vi "Data Collection and Save.vi"(7 "CSM Name":string="Data Collection") -> ()   [LabVIEW 2026, in "Data Collection and Save.lvlib"]
uses:
  Data Collection and Save.lvlib
  Supports/Saving States.ctl
  a89fe48b-4482-43cb-96bd-32483feba248.vi
  115e6d42-36e9-43ba-916e-ce7a01ad014e.vi
  adca8abf-46f5-4539-9d33-3f3b2a323202.vi
  ca7f3cfa-0f2a-41ea-9b26-bce09b64ebef.vi
  b5cc49b7-9397-48e9-91c5-f9ab6ae137c5.vi
  eabdaa19-4c7a-45d4-a202-ab5b619048cc.vi
  94bfd1e9-2896-4ece-95aa-b4a38b10d538.vi
  2868361d-398a-4950-9d8e-d0481113e34b.vi
  74be65fa-d069-47f2-ae0a-2e3cfef6bdd0.vi
  <userlib>/_NEVSTOP/Communicable State Machine(CSM)/AdvanceAPI/CSM - Revert Arguments-Safe String.vi
  <userlib>/_NEVSTOP/Communicable State Machine(CSM)/_Shared/Trim Single-line Text.vi
  <userlib>/_NEVSTOP/Communicable State Machine(CSM)/AdvanceAPI/CSM - Make String Arguments Safe.vi
  <userlib>/_NEVSTOP/Communicable State Machine(CSM)/AdvanceAPI/CSM - Break Down Multiple States String.vi
  <userlib>/_NEVSTOP/Communicable State Machine(CSM)/AdvanceAPI/CSM - Compact Multiple States.vi
  <userlib>/_NEVSTOP/Communicable State Machine(CSM)/AdvanceAPI/CSM - Keywords.vi
  <userlib>/_NEVSTOP/Communicable State Machine(CSM)/addons/API-String-Arugments-Support/_Support/Convert API String Arguments to Data(variant).vi
  <userlib>/_NEVSTOP/Communicable State Machine(CSM)/addons/MassData-Parameter/_support/FGV-MassData(lvlibp).vi
  <vilib>/Utility/file.llb/Write To Spreadsheet File (string).vi
  <vilib>/Utility/file.llb/Write To Spreadsheet File (DBL).vi
  <userlib>/_NEVSTOP/Communicable State Machine(CSM)/Communicable State Machine.lvlib
  <userlib>/_NEVSTOP/Communicable State Machine(CSM)/addons/Loop-Support/CSM Loop Support.lvlib
  <userlib>/_NEVSTOP/Communicable State Machine(CSM)/addons/Logger/CSM File Logger.lvlib
panel:
  in  "Exit":bool
  out "Error Occurred":errorcluster
  out "State History":string
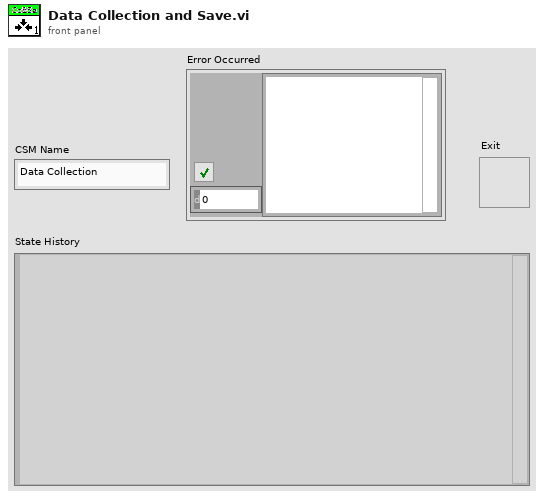
[diagram p1: front panel]
types:
  T1 = enum32{"Invalid", "Standard", "Closed", "Hidden", "Minimized", "Maximized"}
  T2 = enum32{"invalid app kind", "Development System", "Run Time System", "Student Edition", "Embedded LabVIEW", "Evaluation", "Custom"}
  T3 = typedef "温度保存信息.ctl" = cluster{"温度保存-时间":string, "合并保存？":bool, "保存路径":path, "Intervals":dbl}
  T4 = typedef "Data Collection and Save.lvlib/Saving States.ctl" = enum16{"Idle", "Saving", "Error"}
  T5 = typedef "Communicable State Machine.lvlib/_CSM_Response Source Message.ctl" = cluster{"‘State":string, "’Arguments":string, "’Error":errorcluster}
  T6 = cluster{"Current VI Reference":refnum<vi>, "Close Panel on Exit?":bool}
  T7 = typedef "全局变量数据.ctl" = cluster{"温度采集":dbl[], "温度控制":dbl[], "压力测量":dbl[], "Zolix":dbl[], "步进电机":dbl[], "湿度测量":dbl[], "距离测量":dbl[]}
  T8 = cluster{"Core":cluster{"Current VI Reference":refnum<vi>, "Close Panel on Exit?":bool}, "State":T4, "数据及Titles":cluster{"Titles":string[], "温度相关数据":T7}, "文件保存信息":cluster{"温度数据保存文件-时间":string, "合并保存？":bool, "BasePath":path, "Intervals":dbl}, "自停标志":cluster{"接收数":u32, "停止次数":u32, "interval 备份":dbl, "采集时间":timestamp}}
  T9 = cluster{"接收数":u32, "停止次数":u32, "interval 备份":dbl, "采集时间":timestamp}
  T10 = cluster{"温度数据保存文件-时间":string, "合并保存？":bool, "BasePath":path, "Intervals":dbl}
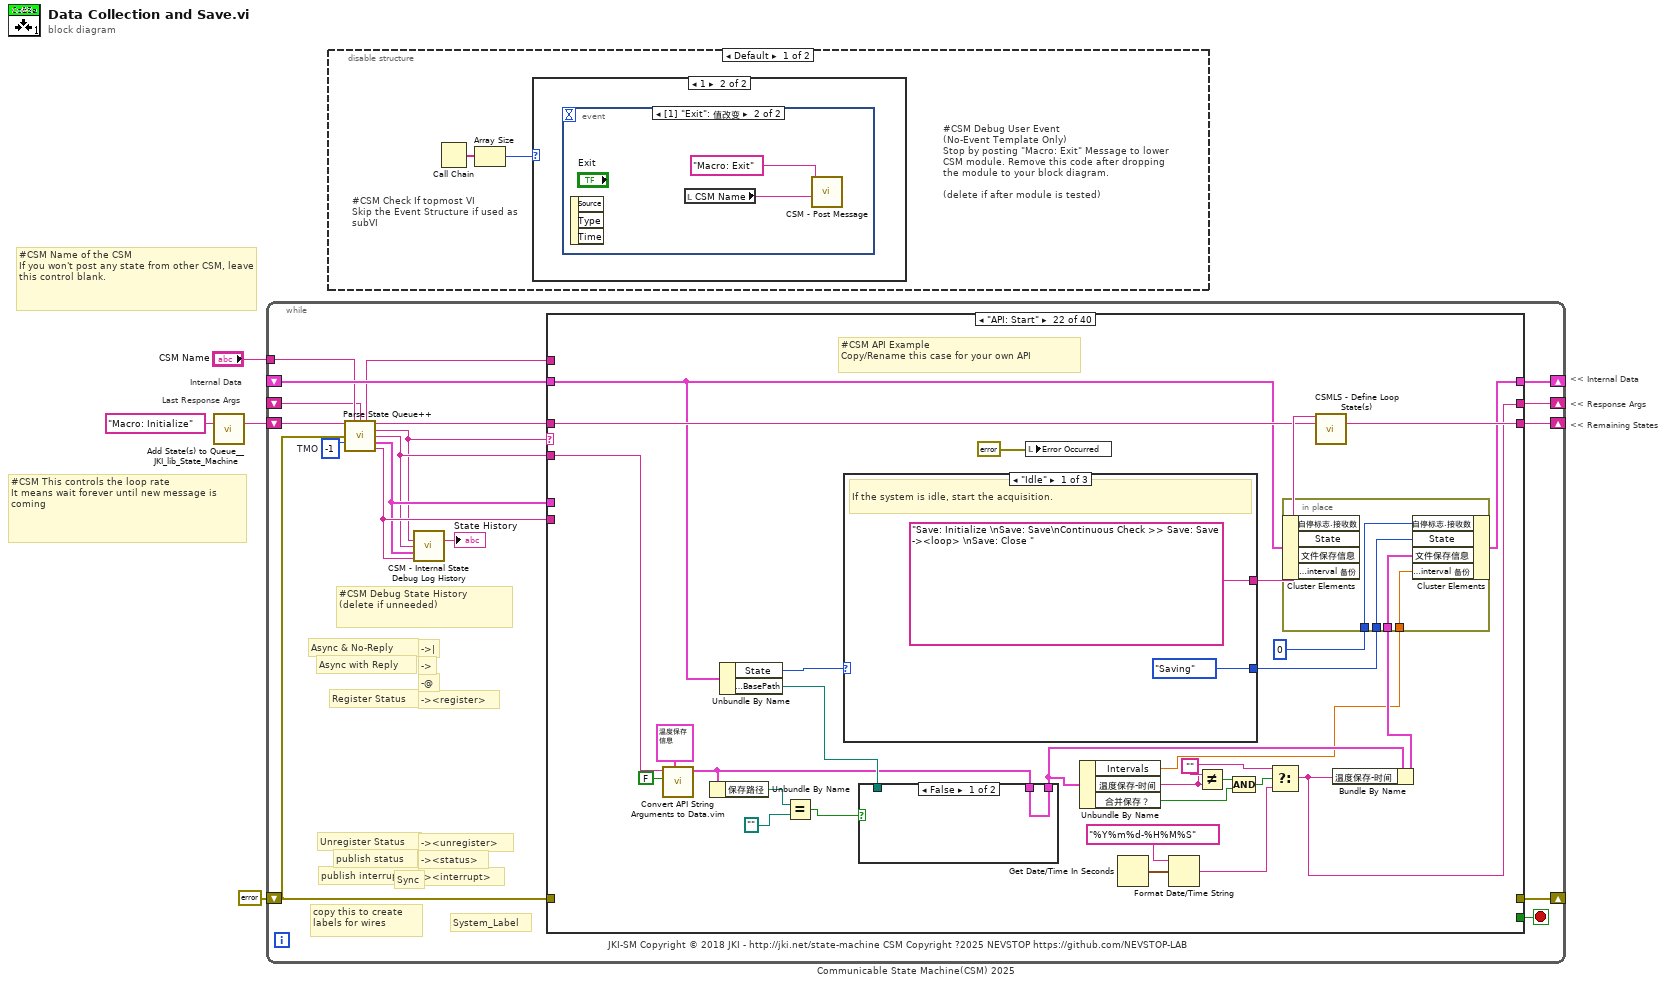
[diagram p0: block diagram]
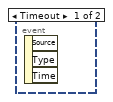
[diagram p3: hidden frame]
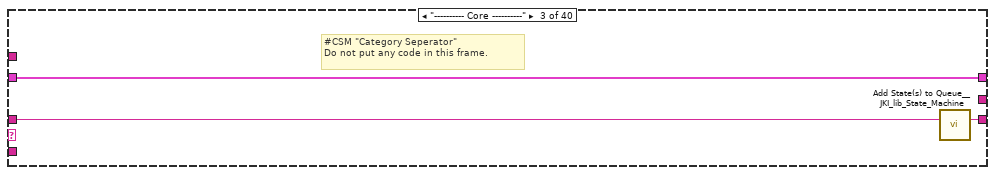
[diagram p7: hidden frame]
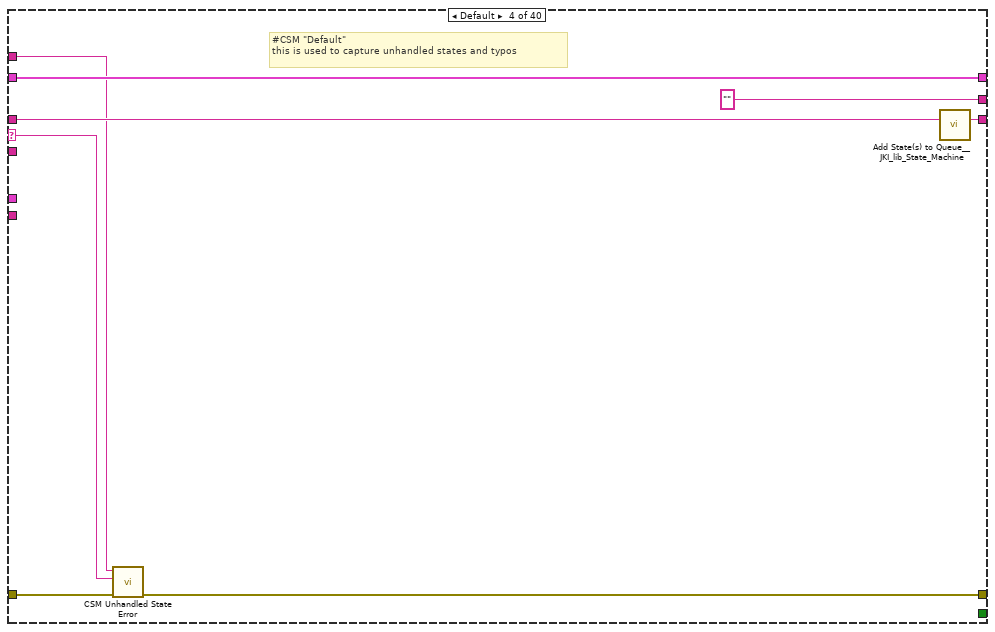
[diagram p8: hidden frame]
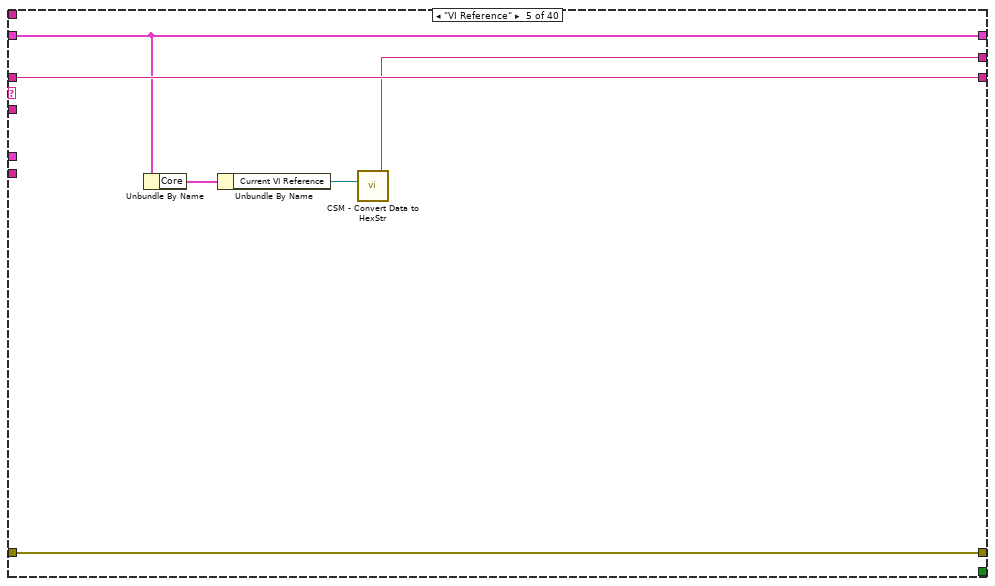
[diagram p9: hidden frame]
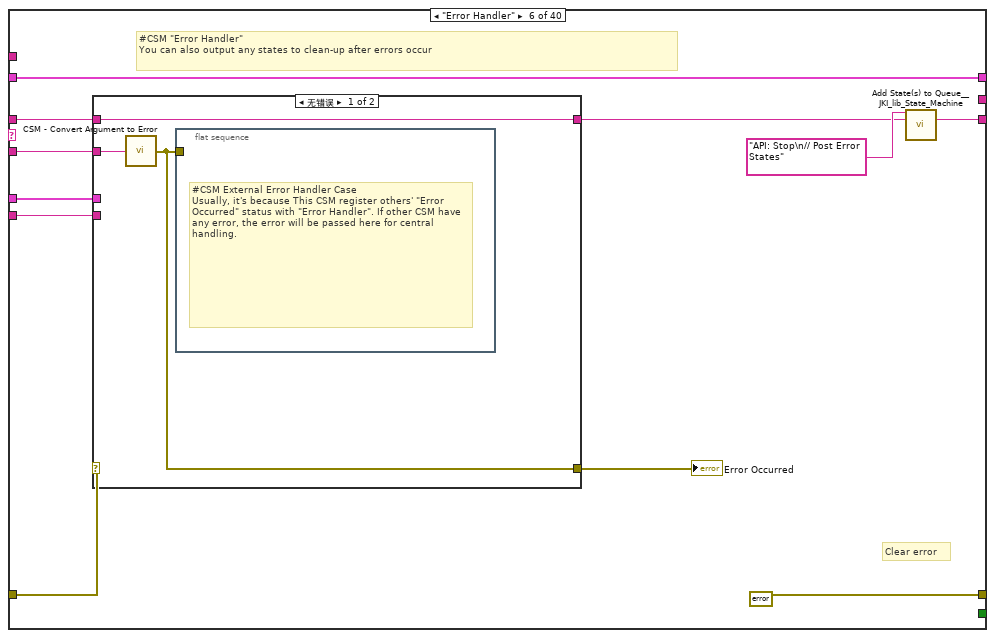
[diagram p10: hidden frame]
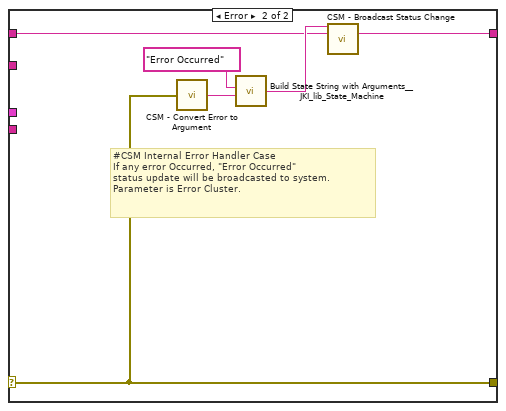
[diagram p11: hidden frame]
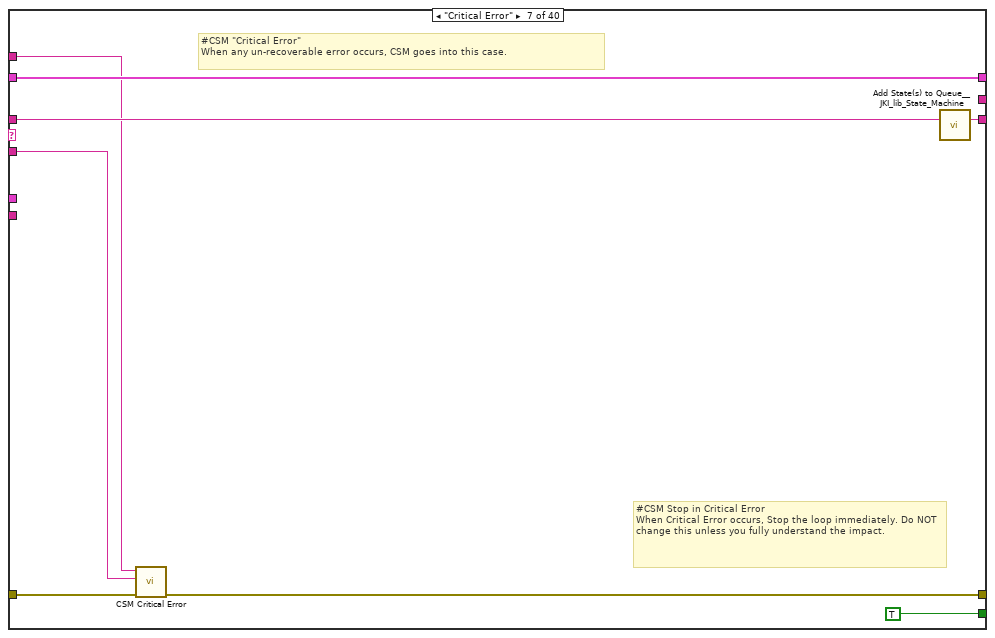
[diagram p12: hidden frame]
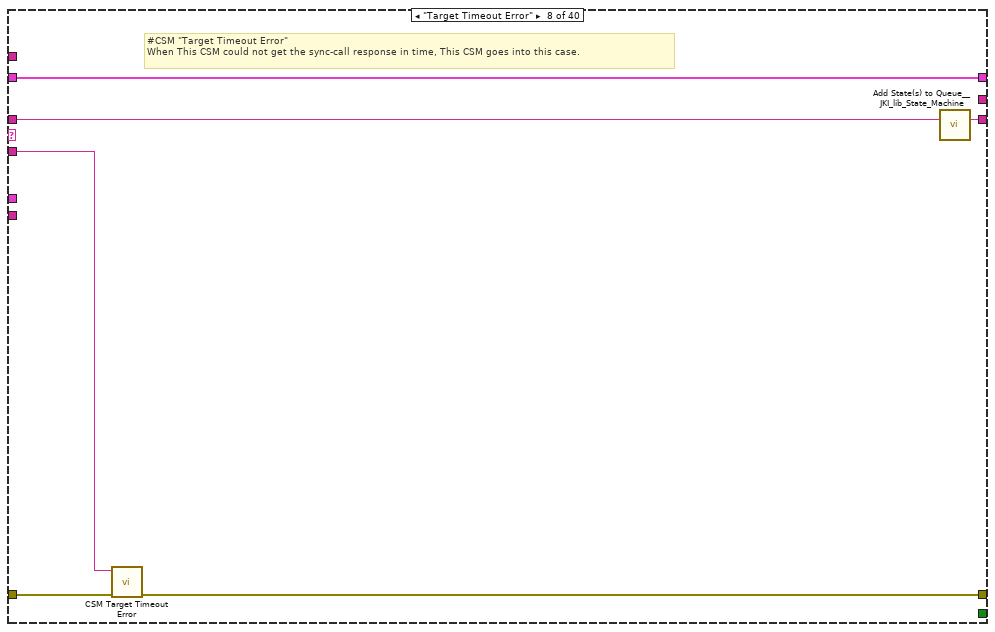
[diagram p13: hidden frame]
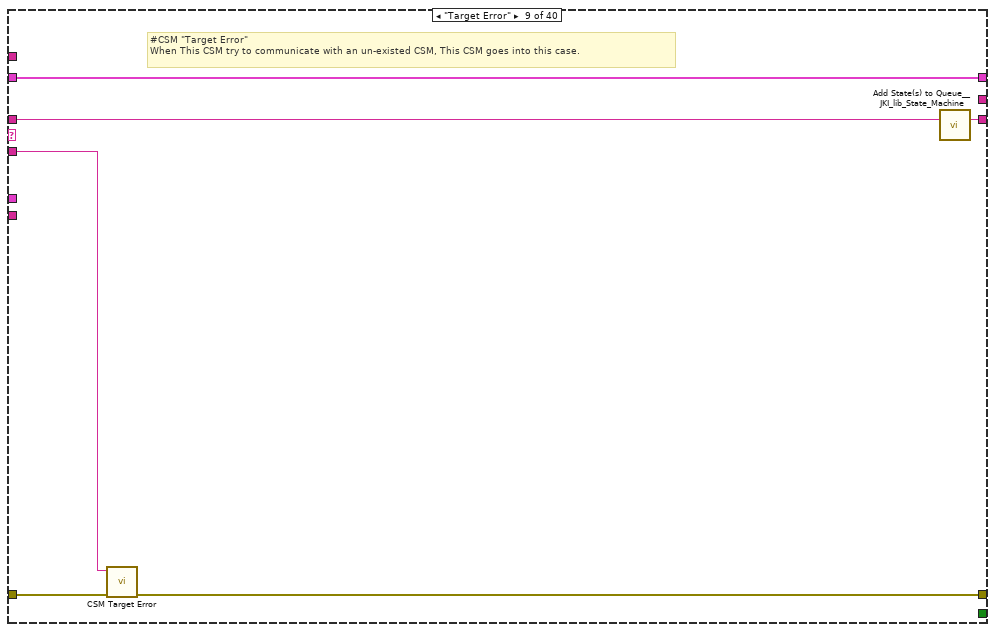
[diagram p14: hidden frame]
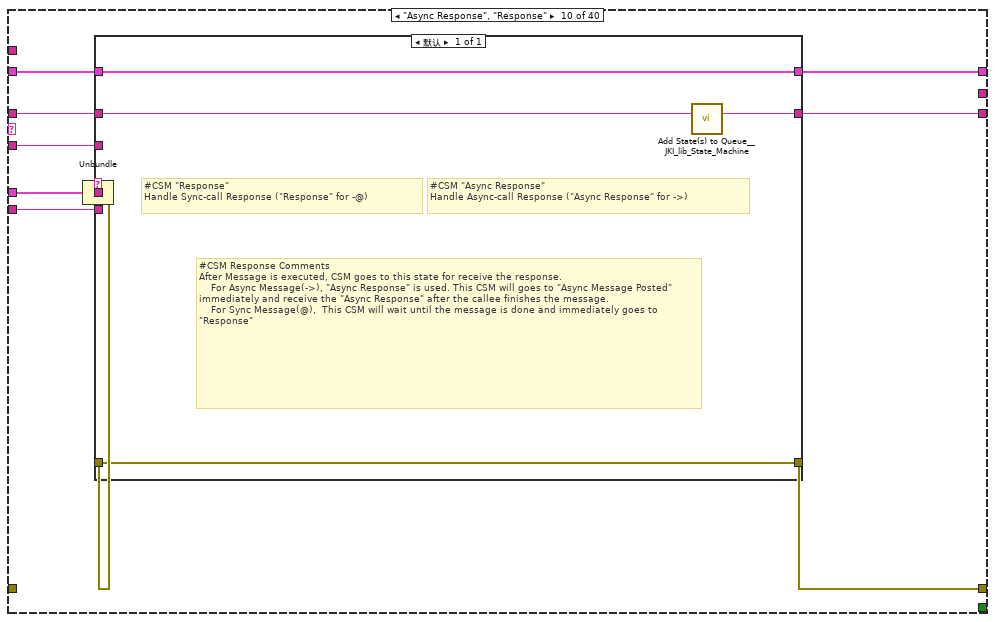
[diagram p15: hidden frame]
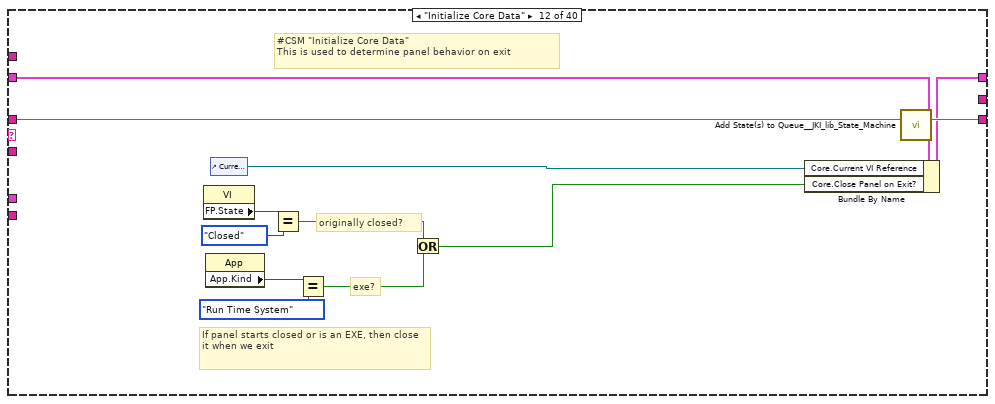
[diagram p17: hidden frame]
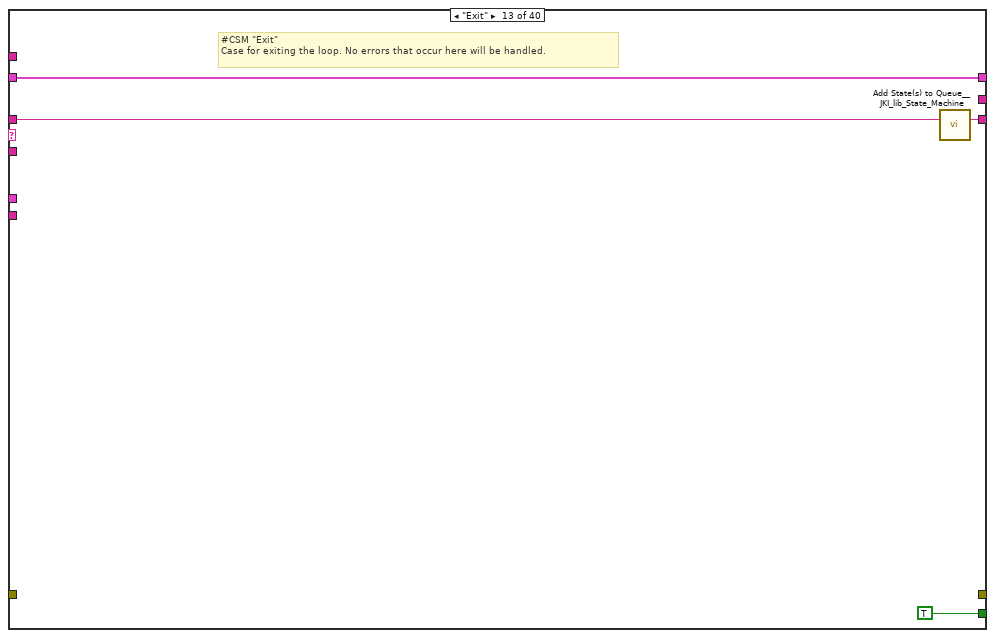
[diagram p18: hidden frame]
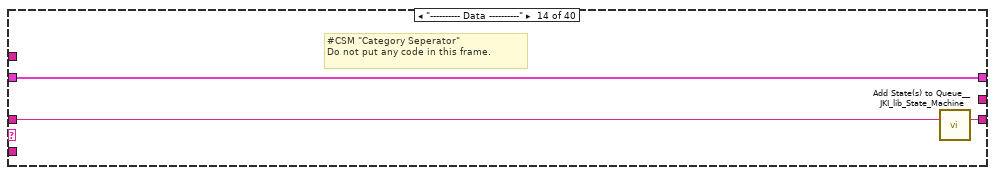
[diagram p19: hidden frame]
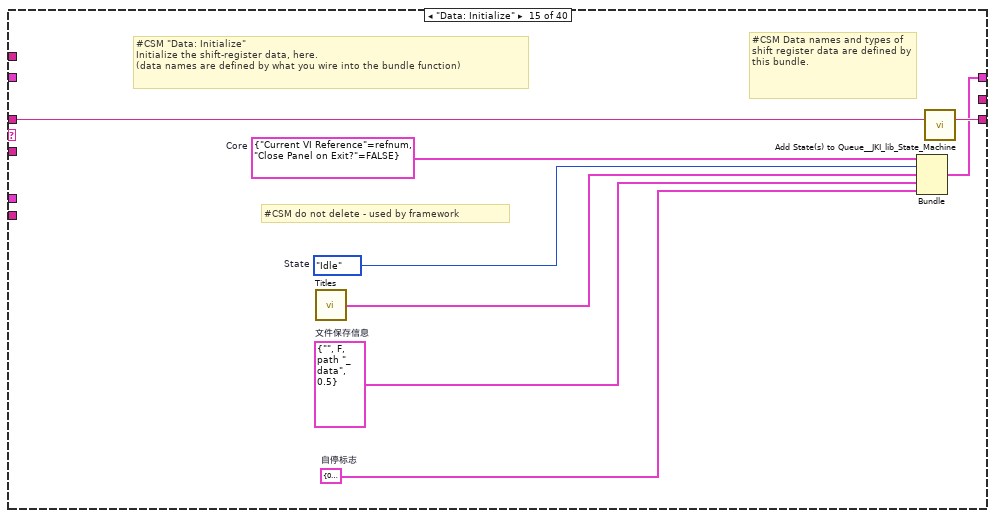
[diagram p20: hidden frame]
diagram:
  # "Last Response Args"
  # "Internal Data"
  # "#CSM Name of the CSM\nIf you won't post any state from other CSM, leave this control blank."
  # "#CSM This controls the loop rate\nIt means wait forever until new message is coming"
  # "<< Internal Data"
  # "<< Response Args"
  # "<< Remaining States"
  n1 = call <vilib>:"Add State(s) to Queue__JKI_lib_State_Machine.vi"("State(s) in (\"\")"="Macro: Initialize" ("Init State(\"Macro: Initialize\")")) -> ("States Out"=w1:string)  [unwired: 14 in]
  n2 = while "Communicable State Machine(CSM) 2025" {
    shift-right: [w17] -> _
    shift-left: _ -> [w16]
    shift-right: [w20] -> _
    shift-left: errorcluster {"status"=FALSE, "code"=0, "source"=""} ("error out") -> [w6]
    shift-right: [w19] -> _
    shift-left: w1 -> [w21]
    tunnel: "CSM Name" -> [w13]
    shift-right: [w14] -> _
    shift-left: _ -> [w8]
    stop <- w18 stop-if-true
    w15 = -1  # TMO
    # "#CSM Debug State History\n(delete if unneeded)"
    # "-><interrupt>"
    # "-><status>"
    # "-><unregister>"
    # "-><register>"
    # "-@"
    # "->"
    # "->|"
    # "publish interrupt"
    # "publish status"
    # "Unregister Status"
    # "Register Status"
    # "Sync"
    # "Async with Reply"
    # "Async & No-Reply"
    # "JKI-SM Copyright © 2018 JKI - http://jki.net/state-machine CSM Copyright ?2025 NEVSTOP https://github.com/NEVSTOP-LAB"
    # "copy this to create labels for wires"
    # "System_Label"
    n3 = call <userlib>:"Parse State Queue++.vi"("State Queue"=w21, "Name (\"\" to Use UUID)"=w13, "Response Arguments"=w8, "Previous Error"=w6, "Dequeue (1 ms)"=w15) -> ("Name Used"=w7:string, "Remaining States"=w22:string, "Current State"=w9:string, "Arguments"=w10:string, "Additional Information"=w11:T5, "Source CSM"=w12:string)  [unwired: 5 in]
    n4 = call <userlib>:"CSM - Internal State Debug Log History.vi"("State"=w9, "Arguments (\"\")"=w10, ">> Response Source Message >>"=w11, "Source (\"\")"=w12) -> ("Debug Log"=→"State History":string)  [unwired: 11 in]
    n5 = case shown="\"API: Start\"" w9 {
      selector: w9 -> [_ _ _ w33 _ _ _ _ _ _ _ _ _ _ _ _ _ _ _ _ _ _ _ _ _ _ _ _ _ _ _ _ _ _ _ _ _ _ w400 _]
      tunnel: w22 -> [w23 w26 w29 w37 w42 w48 w71 w77 w83 w93 w100 w112 w116 w119 w127 w130 w136 w139 w143 w151 w156 w184 w203 w214 w218 w228 w240 w252 w264 w276 w288 w300 w305 w318 w330 w365 w370 w374 w401 w406]
      tunnel: w10 -> [_ _ _ _ _ w47 w67 w74 w80 w87 _ _ _ _ _ _ _ _ _ _ _ w181 _ w212 _ w226 w237 w249 w260 w272 w284 w296 _ _ _ _ _ _ w398 _]
      tunnel: w16 -> [w24 w25 w27 w35 w41 w53 w69 w75 w81 w91 w99 w106 w114 w117 _ w128 w131 w137 w141 w147 w157 w163 w204 w210 w216 w222 w234 w246 w258 w270 w282 w294 w303 w309 w326 w363 w367 w372 w378 w405]
      tunnel: [_ _ _ w30 w43 errorcluster {"status"=FALSE, "code"=0, "source"=""} ("error out") w64 w72 w78 w94 _ _ _ _ _ _ w132 _ _ _ _ _ _ _ _ _ _ _ _ _ _ _ _ w310 w332 _ _ _ _ w407] -> w20
      tunnel: w6 -> [_ _ _ w31 w43 w51 w65 w73 w79 _ _ _ _ _ _ _ w133 _ _ _ _ _ _ _ _ _ _ _ _ _ _ _ _ _ w333 _ _ _ _ w407]
      tunnel: [w23 w26 w28 w36 w42 w49 w70 w76 w82 w92 w100 w111 w115 w118 w126 w130 w135 w138 w142 w150 w155 w183 w202 w213 w217 w227 w239 w251 w263 w275 w287 w299 w304 w318 w331 w364 w369 w373 w399 w404] -> w19
      tunnel: [_ _ _ _ _ _ TRUE _ _ _ _ _ TRUE _ _ _ _ _ _ _ _ _ _ _ _ _ _ _ _ _ _ _ _ _ _ _ _ _ _ _] -> w18
      tunnel: [w24 w25 w27 w35 w41 w53 w69 w75 w81 w90 w99 w110 w114 w117 w125 w128 w131 w137 w141 w147 w157 w162 w204 w209 w216 w221 w233 w245 w257 w269 w281 w291 w303 w308 w329 w363 w366 w372 w377 w405] -> w17
      tunnel: w12 -> [_ _ _ _ _ w46 _ _ _ w88 _ _ _ _ _ _ _ _ _ _ _ _ _ _ _ _ _ _ _ _ _ _ _ _ _ _ _ _ _ _]
      tunnel: w11 -> [_ _ _ _ _ w45 _ _ _ w89 _ _ _ _ _ _ _ _ _ _ _ _ _ _ _ _ _ _ _ _ _ _ _ _ _ _ _ _ _ _]
      tunnel: [_ _ _ "" w38 _ _ _ _ _ _ _ _ _ _ _ _ _ _ _ _ w166 _ _ _ _ _ _ _ _ _ _ _ _ _ _ _ _ _ _] -> w14
      tunnel: w7 -> [_ _ _ w32 _ _ w66 _ _ _ _ _ _ _ _ _ _ _ _ _ _ _ _ _ _ _ _ _ _ _ _ _ _ _ _ _ _ _ _ _]
      frame "", "Idle" {
        # "#CSM \"Idle/Event Handler\"\nexecutes when the state queue is empty"
      }
      frame "CSM Documentation" {
        # "#CSM State Syntax\n\n// Comment line, all text to the right of “//” will be ignored\n// Local Message Example\nDoSth: DoA >> Arguments\n\n// Sync Call Example\nAPI: xxxx >> Arguments -@ TargetModule\n\n// Async Call Example\nAPI: xxxx >> Arguments -> TargetModule\n\n// Async Call without Reply Example\nAPI: xxxx >> Arguments ->| TargetModule\n\n// Broadcast normal status:\nStatus >> StatusArguments  -><status>\n\n// Broadcast Interrupt status:\nInterrupt >> StatusArguments  -><interrupt>\n\n// Register Source Module's status to Handler Module\nStatus@Source Module >> Handler Module@Handler Module -><register>\n\n// Unegister Source Module's status\nStatus@Source Module >> Handler Module -><unregister>"
        # "#CSM README FIRST\n\nCommunicable State Machine(CSM) is a LabVIEW application framework that builds upon JKI State Machine(JKISM). It follows the pattern of JKISM and extends the keywords to describe message communication between modules, including concepts such as Sync-Message, Async-Message, Subscription/Unsubscription of status - essential elements for creating reusable code modules. For more information, please visit the CSM wiki: https://nevstop-lab.github.io/CSM-Wiki/\n\nFor instructions on JKI State Machine, visit: \n    http://jki.net/state-machine/\nFor information about CSM, visit: \n    https://github.com/NEVSTOP-LAB"
        # "#CSM \"Documentation\"\nCase for holding CSM Documenation"
      }
      frame "---------- Core ----------" {
        # "#CSM \"Category Seperator\"\nDo not put any code in this frame."
        n6 = call <vilib>:"Add State(s) to Queue__JKI_lib_State_Machine.vi"("State(s) in (\"\")"=w29) -> ("States Out"=w28:string)  [unwired: 14 in]
      }
      frame Default {
        # "#CSM \"Default\"\nthis is used to capture unhandled states and typos"
        n7 = call <userlib>:"CSM Unhandled State Error.vi"("error in (no error)"=w31, "Undefined State"=w33, "CSM Name"=w32) -> ("error out"=w30:errorcluster)  [unwired: 8 in]
        n8 = call <vilib>:"Add State(s) to Queue__JKI_lib_State_Machine.vi"("State(s) in (\"\")"=w37) -> ("States Out"=w36:string)  [unwired: 14 in]
      }
      frame "VI Reference" {
        n9 = Unbundle By Name(w41) -> ("Core"=w40:T6)
        n10 = Unbundle By Name(w40) -> ("Current VI Reference"=w39:refnum<vi>)
        n11 = call <userlib>:"CSM - Convert Data to HexStr.vi"("Variant"=w39) -> ("HEX String (0-9,A-F)"=w38:string)  [unwired: 8 in]
      }
      frame "Error Handler" {
        # "#CSM \"Error Handler\"\nYou can also output any states to clean-up after errors occur"
        # "Clear error"
        n12 = case shown="无错误" w51 {
          selector: w51 -> [_ w58]
          tunnel: [w57 w60] -> w50
          tunnel: w48 -> [w57 w59]
          tunnel: w47 -> [w56 _]
          tunnel: w46 -> [_ _]
          tunnel: w45 -> [_ _]
          tunnel: [w55 w58] -> w44
          frame No Error {
            n13 = call <userlib>:"CSM - Convert Argument to Error.vi"("Argument"=w56) -> ("Error"=w55:errorcluster)  [unwired: 4 in]
            n14 = flat-sequence {
              tunnel: w55 -> [_]
              frame #0 {
                # "#CSM External Error Handler Case\nUsually, it's because This CSM register others' \"Error Occurred\" status with \"Error Handler\". If other CSM have any error, the error will be passed here for central handling."
              }
            }
          }
          frame Error {
            # "#CSM Internal Error Handler Case \nIf any error Occurred, \"Error Occurred\" \nstatus update will be broadcasted to system.\nParameter is Error Cluster."
            n15 = call <userlib>:"CSM - Convert Error to Argument.vi"("Error"=w58) -> ("Argument"=w62:string)  [unwired: 4 in]
            n16 = call <vilib>:"Build State String with Arguments__JKI_lib_State_Machine.vi"("Arguments (\"\")"=w62, "State"="Error Occurred" ("Status with Arguments")) -> ("State with Arguments"=w61:string)  [unwired: 4 in]
            n17 = call <userlib>:"CSM - Broadcast Status Change.vi"("Status With Arguments"=w61, "State Queue"=w59) -> ("Remaining States"=w60:string)  [unwired: 13 in]
          }
        }
        "Error Occurred" <- w44
        n18 = call <vilib>:"Add State(s) to Queue__JKI_lib_State_Machine.vi"("State(s) in Front (\"\")"="API: Stop\n// Post Error States", "State(s) in (\"\")"=w50) -> ("States Out"=w49:string)  [unwired: 13 in]
      }
      frame "Critical Error" {
        # "#CSM \"Critical Error\"\nWhen any un-recoverable error occurs, CSM goes into this case."
        # "#CSM Stop in Critical Error\nWhen Critical Error occurs, Stop the loop immediately. Do NOT change this unless you fully understand the impact."
        n19 = call <userlib>:"CSM Critical Error.vi"("error in (no error)"=w65, "Arugments (As Reason)"=w67, "CSM Name"=w66) -> ("error out"=w64:errorcluster)  [unwired: 8 in]
        n20 = call <vilib>:"Add State(s) to Queue__JKI_lib_State_Machine.vi"("State(s) in (\"\")"=w71) -> ("States Out"=w70:string)  [unwired: 14 in]
      }
      frame "Target Timeout Error" {
        # "#CSM \"Target Timeout Error\"\nWhen This CSM could not get the sync-call response in time, This CSM goes into this case."
        n21 = call <userlib>:"CSM Target Timeout Error.vi"("error in (no error)"=w73, "Arguments (As CSM Name)"=w74) -> ("error out"=w72:errorcluster)  [unwired: 9 in]
        n22 = call <vilib>:"Add State(s) to Queue__JKI_lib_State_Machine.vi"("State(s) in (\"\")"=w77) -> ("States Out"=w76:string)  [unwired: 14 in]
      }
      frame "Target Error" {
        # "#CSM \"Target Error\"\nWhen This CSM try to communicate with an un-existed CSM, This CSM goes into this case."
        n23 = call <userlib>:"CSM Target Error.vi"("error in (no error)"=w79, "Arguments (As CSM Name)"=w80) -> ("error out"=w78:errorcluster)  [unwired: 9 in]
        n24 = call <vilib>:"Add State(s) to Queue__JKI_lib_State_Machine.vi"("State(s) in (\"\")"=w83) -> ("States Out"=w82:string)  [unwired: 14 in]
      }
      frame "Async Response", "Response" {
        n25 = Unbundle(w89) -> ("‘State"=w86:string, "’Arguments"=w85:string, "’Error"=w84:errorcluster)
        n26 = case shown="默认" w86 {
          tunnel: [w95] -> w92
          tunnel: w93 -> [w96]
          tunnel: [w98] -> w90
          tunnel: w91 -> [w98]
          tunnel: [w97] -> w94
          tunnel: w84 -> [w97]
          tunnel: w88 -> [_]
          tunnel: w87 -> [_]
          tunnel: w85 -> [_]
          frame 默认 {
            # "#CSM \"Async Response\"\nHandle Async-call Response (\"Async Response\" for ->)"
            # "#CSM \"Response\"\nHandle Sync-call Response (\"Response\" for -@)"
            # "#CSM Response Comments\nAfter Message is executed, CSM goes to this state for receive the response.\n    For Async Message(->), \"Async Response\" is used. This CSM will goes to \"Async Message Posted\" immediately and receive the \"Async Response\" after the callee finishes the message.\n    For Sync Message(@),  This CSM will wait until the message is done and immediately goes to \"Response\""
            n27 = call <vilib>:"Add State(s) to Queue__JKI_lib_State_Machine.vi"("State(s) in (\"\")"=w96) -> ("States Out"=w95:string)  [unwired: 14 in]
          }
        }
      }
      frame "Async Message Posted" {
        # "#CSM \"Async Message Posted\"\nAfter Async Message is posted (-> or ->| ), CSM goes to this state for post-action.\nYou can use Argument - State to tell which Async Message is called."
      }
      frame "Initialize Core Data" {
        # "#CSM \"Initialize Core Data\"\nThis is used to determine panel behavior on exit"
        # "originally closed?"
        # "exe?"
        # "If panel starts closed or is an EXE, then close it when we exit"
        n28 = property class="VI"() -> ("FP.State"=w103:T1)  [unwired: 2 in, 2 out]
        n29 = property class="App"() -> ("App.Kind"=w109:T2)  [unwired: 2 in, 2 out]
        n30 = control-ref of="Current VI Reference"() -> (w104:refnum<vi>)
        n31 = Equal?(x=w103, y=T1."Closed" ("Front Panel Window:State")) -> (x = y?=w101:bool)
        n32 = Equal?(x=w109, y=T2."Run Time System" ("Application:Kind")) -> (x = y?=w107:bool)
        n33 = Or(x=w101, y=w107) -> (x .or. y?=w105:bool)
        n34 = Bundle By Name(cluster=w106, "Core.Current VI Reference"=w104, "Core.Close Panel on Exit?"=w105) -> (w110:T8)
        n35 = call <vilib>:"Add State(s) to Queue__JKI_lib_State_Machine.vi"("State(s) in (\"\")"=w112) -> ("States Out"=w111:string)  [unwired: 14 in]
      }
      frame "Exit" {
        # "#CSM \"Exit\"\nCase for exiting the loop. No errors that occur here will be handled."
        n36 = call <vilib>:"Add State(s) to Queue__JKI_lib_State_Machine.vi"("State(s) in (\"\")"=w116) -> ("States Out"=w115:string)  [unwired: 14 in]
      }
      frame "---------- Data ----------" {
        # "#CSM \"Category Seperator\"\nDo not put any code in this frame."
        n37 = call <vilib>:"Add State(s) to Queue__JKI_lib_State_Machine.vi"("State(s) in (\"\")"=w119) -> ("States Out"=w118:string)  [unwired: 14 in]
      }
      frame "Data: Initialize" {
        w120 = T9 {"接收数"=0, "停止次数"=0, "interval 备份"=0.0, "采集时间"=timestamp(0 s since 1904-01-01)}  # 自停标志
        w122 = T10 {"温度数据保存文件-时间"="", "合并保存？"=FALSE, "BasePath"=path "_data", "Intervals"=0.5}  # 文件保存信息
        w123 = Saving_States."Idle"  # State
        w124 = T6 {"Current VI Reference"=refnum, "Close Panel on Exit?"=FALSE}  # Core
        # "#CSM \"Data: Initialize\"\nInitialize the shift-register data, here.\n(data names are defined by what you wire into the bundle function)"
        # "#CSM do not delete - used by framework"
        # "#CSM Data names and types of shift register data are defined by this bundle."
        n38 = call "Titles.vi"() -> ("数据及Titles"=w121:cluster{"Titles":string[], "温度相关数据":T7})  [unwired: 1 in]
        n39 = Bundle("Core"=w124, "State"=w123, "数据及Titles"=w121, "文件保存信息"=w122, "自停标志"=w120) -> (w125:T8)  [unwired: 1 in]
        n40 = call <vilib>:"Add State(s) to Queue__JKI_lib_State_Machine.vi"("State(s) in (\"\")"=w127) -> ("States Out"=w126:string)  [unwired: 14 in]
      }
      frame "Data: Update Indicators" {
        n41 = local write "Error Occurred"(errorcluster {"status"=FALSE, "code"=0, "source"=""} ("错误常量")) -> ()
      }
      frame "Data: Cleanup" {
        # "#CSM \"Data: Cleanup\"\nCleanup any data and references, here.\n(this is called automatically, by the Macro: Exit)"
        n42 = Unbundle By Name(w131) -> ("Core.Current VI Reference"=w134:refnum<vi>)
        n43 = Close Reference(reference=w134, error in (no error)=w133) -> (error out=w132:errorcluster)
        n44 = call <vilib>:"Add State(s) to Queue__JKI_lib_State_Machine.vi"("State(s) in (\"\")"=w136) -> ("States Out"=w135:string)  [unwired: 14 in]
      }
      frame "---------- Macro ----------" {
        # "#CSM \"Category Seperator\"\nDo not put any code in this frame."
        n45 = call <vilib>:"Add State(s) to Queue__JKI_lib_State_Machine.vi"("State(s) in (\"\")"=w139) -> ("States Out"=w138:string)  [unwired: 14 in]
      }
      frame "Macro: Initialize" {
        # "#CSM \"Macro: Initialize\"\nInitialization Macro (This is called once, when the VI starts)"
        n46 = call <vilib>:"Add State(s) to Queue__JKI_lib_State_Machine.vi"("State(s) in Front (\"\")"="Data: Initialize\nInitialize Core Data\nData: Update Indicators", "State(s) in (\"\")"=w143) -> ("States Out"=w142:string)  [unwired: 13 in]
      }
      frame "Macro: Exit" {
        # "#CSM \"Macro: Exit\"\nExit Macro (This is called once, when the VI exits)"
        n47 = Unbundle By Name(w147) -> ("State"=w146:T4)
        n48 = case shown="\"Saving\"" w146 {
          tunnel: ["" "Break Continuous\nDAQ: Close" ""] -> w144
          frame "Idle", Default {
          }
          frame "Saving" {
          }
          frame "Error" {
          }
        }
        n49 = call <vilib>:"Add State(s) to Queue__JKI_lib_State_Machine.vi"("State(s) in Front (\"\")"="//Exit Sub-Modules ", "State(s) in (\"\")"=w144, "State(s) at Back (\"\")"="Data: Cleanup\nExit") -> ("States Out"=w148:string)  [unwired: 12 in]
        n50 = call <vilib>:"Add State(s) to Queue__JKI_lib_State_Machine.vi"("State(s) in Front (\"\")"=w148, "State(s) in (\"\")"=w151) -> ("States Out"=w150:string)  [unwired: 13 in]
      }
      frame "---------- API ----------" {
        # "#CSM \"Category Seperator\"\nDo not put any code in this frame."
        n51 = call <vilib>:"Add State(s) to Queue__JKI_lib_State_Machine.vi"("State(s) in (\"\")"=w156) -> ("States Out"=w155:string)  [unwired: 14 in]
      }
      frame "API: Start" {
        # "#CSM API Example\nCopy/Rename this case for your own API"
        n52 = call "Convert API String Arguments to Data.vim"("Reference Type"=T3 {"温度保存-时间"="", "合并保存？"=FALSE, "保存路径"=path "D:/sunrise/data", "Intervals"=0.0} ("输出簇"), "Strict Label Check? (T)"=FALSE, "API String"=w181) -> ("Data"=w176:T3)  [unwired: 5 in, 1 out]
        n53 = Unbundle By Name(w176) -> ("保存路径"=w179:path)
        n54 = Unbundle By Name(w163) -> ("State"=w186:T4, "文件保存信息.BasePath"=w178:path)
        n55 = Equal?(x=w179, y=path "") -> (x = y?=w177:bool)
        n56 = case shown="\"Idle\"" w186 {
          selector: w186 -> [_ w199 w200]
          tunnel: [Saving_States."Saving" ("Acquisition State") w199 w200] -> w160
          tunnel: ["Save: Initialize \nSave: Save\nContinuous Check >> Save: Save -><loop> \nSave: Close " ("State(s) in Front (\"\")") _ _] -> w185
          frame "Idle" {
            # "If the system is idle, start the acquisition."
          }
          frame "Saving" {
            # "The system is already acquiring. Ignore the \"Start\" message."
          }
          frame "Error" {
          }
        }
        n57 = case shown="False" w177 {
          tunnel: w178 -> [_ w196]
          tunnel: w176 -> [w191 w195]
          tunnel: [w191 w194] -> w167
          frame False {
          }
          frame True {
            n58 = call <userlib>:"Append CSM AppDir If Relative.vi"("Relative Path (.)"=w196) -> ("Application Directory (+ Relative)"=w193:path)  [unwired: 4 in]
            n59 = call "__MGI Create Directory Chain_CO.vi"("Path"=w193) -> ("Duplicate Path"=w192:path)  [unwired: 9 in, 1 out]
            n60 = Bundle By Name(cluster=w195, "保存路径"=w192) -> (w194:T3)
          }
        }
        n61 = local write "Error Occurred"(errorcluster {"status"=FALSE, "code"=0, "source"=""} ("错误常量")) -> ()
        n62 = Unbundle By Name(w167) -> ("Intervals"=w158:dbl, "温度保存-时间"=w169:string, "合并保存？"=w168:bool)
        n63 = Get Date/Time In Seconds() -> (seconds since 1Jan1904=w173:timestamp)
        n64 = Format Date/Time String(time format string (%c)="%Y%m%d-%H%M%S" ("时间格式字符串(%c)"), seconds (now)=w173) -> (date/time string=w170:string)  [unwired: 1 in]
        n65 = Not Equal?(x="", y=w169) -> (x != y?=w174:bool)
        n66 = Compound Arithmetic op=AND ("复合运算")(w174, w168) -> (w175:bool)
        n67 = Select(t=w169, s=w175, f=w170) -> (s? t:f=w166:string)
        n68 = call <userlib>:"CSMLS - Define Loop State(s).vi"("Loop States"=w185, "States Queue"=w184) -> ("Remaining States"=w183:string)  [unwired: 13 in]
        n69 = Bundle By Name(cluster=w167, "温度保存-时间"=w166) -> (w159:T3)
        n70 = in-place {
          in-place-border: u32 0 ("广播数") -> [w190]
          in-place-border: w160 -> [w189]
          in-place-border: w159 -> [w188]
          in-place-border: w158 -> [w187]
          n71 = in-place-cluster #1(w163) -> ()  [unwired: 4 out]
          n72 = in-place-cluster #1("自停标志.接收数"=w190, "State"=w189, "文件保存信息"=w188, "自停标志.interval 备份"=w187) -> (w162:T8)
        }
      }
      frame "API: Stop" {
        # "#CSM API Example\nCopy/Rename this case for your own API"
        n73 = Unbundle By Name(w204) -> ("State"=w205:T4)
        n74 = case shown="\"Saving\"" w205 {
          tunnel: [_ "Break Continuous" ("State(s) in Front (\"\")") "Break Continuous" ("State(s) in Front (\"\")")] -> w201
          frame "Idle" {
            # "The system is already idle. Ignore the \"Stop\" message."
          }
          frame "Saving" {
            # "If the system is acquiring, stop the acquisition."
          }
          frame "Error" {
          }
        }
        n75 = call <vilib>:"Add State(s) to Queue__JKI_lib_State_Machine.vi"("State(s) in Front (\"\")"=w201, "State(s) in (\"\")"=w203) -> ("States Out"=w202:string)  [unwired: 13 in]
      }
      frame "API: Save Interval" {
        n76 = call "Convert API String Arguments to Data.vim"("Reference Type"=0.0, "API String"=w212) -> ("Data"=w208:dbl)  [unwired: 6 in, 1 out]
        n77 = in-place {
          in-place-border: w208 -> [w215]
          n78 = in-place-cluster #2(w210) -> ()  [unwired: 2 out]
          n79 = in-place-cluster #2("文件保存信息.Intervals"=w215, "自停标志.interval 备份"=w215) -> (w209:T8)
        }
        n80 = call <vilib>:"Add State(s) to Queue__JKI_lib_State_Machine.vi"("State(s) in (\"\")"=w214) -> ("States Out"=w213:string)  [unwired: 14 in]
      }
      frame "---------- Collection ----------" {
        # "#CSM \"Category Seperator\"\nDo not put any code in this frame."
        n81 = call <vilib>:"Add State(s) to Queue__JKI_lib_State_Machine.vi"("State(s) in (\"\")"=w218) -> ("States Out"=w217:string)  [unwired: 14 in]
      }
      frame "Coll: TP1" {
        w224 = cluster{"采集时间":timestamp, "Data":dbl[]} {"采集时间"=timestamp(0 s since 1904-01-01), "Data"=[]}  # Time and Data
        # "#CSM \"Category Seperator\"\nDo not put any code in this frame."
        n82 = call "CSM - Convert Argument to MassData.vim"("Type"=w224, "MassData Argument"=w226) -> ("Data"=w225:cluster{"采集时间":timestamp, "Data":dbl[]})  [unwired: 6 in, 1 out]
        n83 = Unbundle By Name(w222) -> ("自停标志.接收数"=w223:u32)
        n84 = Unbundle By Name(w225) -> ("Data"=w219:dbl[])
        n85 = Increment(x=w223) -> (x+1=w220:u32)
        n86 = in-place {
          in-place-border: w220 -> [w230]
          in-place-border: w219 -> [w229]
          n87 = in-place-cluster #3(w222) -> ()  [unwired: 2 out]
          n88 = in-place-cluster #3("自停标志.接收数"=w230, "数据及Titles.温度相关数据.温度采集"=w229) -> (w221:T8)
        }
        n89 = call <vilib>:"Add State(s) to Queue__JKI_lib_State_Machine.vi"("State(s) in (\"\")"=w228) -> ("States Out"=w227:string)  [unwired: 14 in]
      }
      frame "Coll: WK1" {
        w236 = cluster{"采集时间":timestamp, "Data":dbl[]} {"采集时间"=timestamp(0 s since 1904-01-01), "Data"=[]}  # Time and Data
        # "#CSM \"Category Seperator\"\nDo not put any code in this frame."
        n90 = Unbundle By Name(w234) -> ("自停标志.接收数"=w235:u32)
        n91 = call "CSM - Convert Argument to MassData.vim"("Type"=w236, "MassData Argument"=w237) -> ("Data"=w238:cluster{"采集时间":timestamp, "Data":dbl[]})  [unwired: 6 in, 1 out]
        n92 = Increment(x=w235) -> (x+1=w232:u32)
        n93 = Unbundle By Name(w238) -> ("Data"=w231:dbl[])
        n94 = in-place {
          in-place-border: w232 -> [w242]
          in-place-border: w231 -> [w241]
          n95 = in-place-cluster #4(w234) -> ()  [unwired: 2 out]
          n96 = in-place-cluster #4("自停标志.接收数"=w242, "数据及Titles.温度相关数据.温度控制"=w241) -> (w233:T8)
        }
        n97 = call <vilib>:"Add State(s) to Queue__JKI_lib_State_Machine.vi"("State(s) in (\"\")"=w240) -> ("States Out"=w239:string)  [unwired: 14 in]
      }
      frame "Coll: PS1" {
        w250 = cluster{"采集时间":timestamp, "Data":dbl[]} {"采集时间"=timestamp(0 s since 1904-01-01), "Data"=[]}  # Time and Data
        # "#CSM \"Category Seperator\"\nDo not put any code in this frame."
        n98 = Unbundle By Name(w246) -> ("自停标志.接收数"=w247:u32)
        n99 = call "CSM - Convert Argument to MassData.vim"("Type"=w250, "MassData Argument"=w249) -> ("Data"=w248:cluster{"采集时间":timestamp, "Data":dbl[]})  [unwired: 6 in, 1 out]
        n100 = Unbundle By Name(w248) -> ("Data"=w243:dbl[])
        n101 = Increment(x=w247) -> (x+1=w244:u32)
        n102 = in-place {
          in-place-border: w244 -> [w254]
          in-place-border: w243 -> [w253]
          n103 = in-place-cluster #5(w246) -> ()  [unwired: 2 out]
          n104 = in-place-cluster #5("自停标志.接收数"=w254, "数据及Titles.温度相关数据.压力测量"=w253) -> (w245:T8)
        }
        n105 = call <vilib>:"Add State(s) to Queue__JKI_lib_State_Machine.vi"("State(s) in (\"\")"=w252) -> ("States Out"=w251:string)  [unwired: 14 in]
      }
      frame "Coll: ZO1" {
        w262 = cluster{"采集时间":timestamp, "Data":dbl[]} {"采集时间"=timestamp(0 s since 1904-01-01), "Data"=[]}  # Time and Data
        # "#CSM \"Category Seperator\"\nDo not put any code in this frame."
        n106 = Unbundle By Name(w258) -> ("自停标志.接收数"=w259:u32)
        n107 = call "CSM - Convert Argument to MassData.vim"("Type"=w262, "MassData Argument"=w260) -> ("Data"=w261:cluster{"采集时间":timestamp, "Data":dbl[]})  [unwired: 6 in, 1 out]
        n108 = Unbundle By Name(w261) -> ("Data"=w255:dbl[])
        n109 = Increment(x=w259) -> (x+1=w256:u32)
        n110 = in-place {
          in-place-border: w256 -> [w266]
          in-place-border: w255 -> [w265]
          n111 = in-place-cluster #6(w258) -> ()  [unwired: 2 out]
          n112 = in-place-cluster #6("自停标志.接收数"=w266, "数据及Titles.温度相关数据.Zolix"=w265) -> (w257:T8)
        }
        n113 = call <vilib>:"Add State(s) to Queue__JKI_lib_State_Machine.vi"("State(s) in (\"\")"=w264) -> ("States Out"=w263:string)  [unwired: 14 in]
      }
      frame "Coll: MO1" {
        w274 = cluster{"采集时间":timestamp, "Data":dbl[]} {"采集时间"=timestamp(0 s since 1904-01-01), "Data"=[]}  # Time and Data
        # "#CSM \"Category Seperator\"\nDo not put any code in this frame."
        n114 = Unbundle By Name(w270) -> ("自停标志.接收数"=w271:u32)
        n115 = call "CSM - Convert Argument to MassData.vim"("Type"=w274, "MassData Argument"=w272) -> ("Data"=w273:cluster{"采集时间":timestamp, "Data":dbl[]})  [unwired: 6 in, 1 out]
        n116 = Unbundle By Name(w273) -> ("Data"=w267:dbl[])
        n117 = Increment(x=w271) -> (x+1=w268:u32)
        n118 = in-place {
          in-place-border: w268 -> [w278]
          in-place-border: w267 -> [w277]
          n119 = in-place-cluster #7(w270) -> ()  [unwired: 2 out]
          n120 = in-place-cluster #7("自停标志.接收数"=w278, "数据及Titles.温度相关数据.步进电机"=w277) -> (w269:T8)
        }
        n121 = call <vilib>:"Add State(s) to Queue__JKI_lib_State_Machine.vi"("State(s) in (\"\")"=w276) -> ("States Out"=w275:string)  [unwired: 14 in]
      }
      frame "Coll: HM1" {
        w286 = cluster{"采集时间":timestamp, "Data":dbl[]} {"采集时间"=timestamp(0 s since 1904-01-01), "Data"=[]}  # Time and Data
        # "#CSM \"Category Seperator\"\nDo not put any code in this frame."
        n122 = Unbundle By Name(w282) -> ("自停标志.接收数"=w283:u32)
        n123 = call "CSM - Convert Argument to MassData.vim"("Type"=w286, "MassData Argument"=w284) -> ("Data"=w285:cluster{"采集时间":timestamp, "Data":dbl[]})  [unwired: 6 in, 1 out]
        n124 = Unbundle By Name(w285) -> ("Data"=w279:dbl[])
        n125 = Increment(x=w283) -> (x+1=w280:u32)
        n126 = in-place {
          in-place-border: w280 -> [w290]
          in-place-border: w279 -> [w289]
          n127 = in-place-cluster #8(w282) -> ()  [unwired: 2 out]
          n128 = in-place-cluster #8("自停标志.接收数"=w290, "数据及Titles.温度相关数据.湿度测量"=w289) -> (w281:T8)
        }
        n129 = call <vilib>:"Add State(s) to Queue__JKI_lib_State_Machine.vi"("State(s) in (\"\")"=w288) -> ("States Out"=w287:string)  [unwired: 14 in]
      }
      frame "Coll: DS1" {
        w298 = cluster{"采集时间":timestamp, "Data":dbl[]} {"采集时间"=timestamp(0 s since 1904-01-01), "Data"=[]}  # Time and Data
        # "#CSM \"Category Seperator\"\nDo not put any code in this frame."
        n130 = Unbundle By Name(w294) -> ("自停标志.接收数"=w295:u32)
        n131 = call "CSM - Convert Argument to MassData.vim"("Type"=w298, "MassData Argument"=w296) -> ("Data"=w297:cluster{"采集时间":timestamp, "Data":dbl[]})  [unwired: 6 in, 1 out]
        n132 = Unbundle By Name(w297) -> ("Data"=w292:dbl[])
        n133 = Increment(x=w295) -> (x+1=w293:u32)
        n134 = in-place {
          in-place-border: w293 -> [w302]
          in-place-border: w292 -> [w301]
          n135 = in-place-cluster #9(w294) -> ()  [unwired: 2 out]
          n136 = in-place-cluster #9("自停标志.接收数"=w302, "数据及Titles.温度相关数据.距离测量"=w301) -> (w291:T8)
        }
        n137 = call <vilib>:"Add State(s) to Queue__JKI_lib_State_Machine.vi"("State(s) in (\"\")"=w300) -> ("States Out"=w299:string)  [unwired: 14 in]
      }
      frame "---------- Save ----------" {
        # "#CSM \"Category Seperator\"\nDo not put any code in this frame."
        n138 = call <vilib>:"Add State(s) to Queue__JKI_lib_State_Machine.vi"("State(s) in (\"\")"=w305) -> ("States Out"=w304:string)  [unwired: 14 in]
      }
      frame "Save: Initialize" {
        # "#CSM \"Category Seperator\"\nDo not put any code in this frame."
        n139 = Unbundle By Name(w309) -> ("文件保存信息.BasePath"=w311:path, "文件保存信息.温度数据保存文件-时间"=w307:string, "数据及Titles.Titles"=w312:string[])
        n140 = Concatenate Strings("温度" ("字符串"), w307, "_T1.dat" ("字符串")) -> (w315:string)
        n141 = Build Path(base path=w311, name or relative path=w315) -> (appended path=w316:path)
        n142 = call <vilib>:"Check if File or Folder Exists.vi"("path"=w316) -> ("error out"=w310:errorcluster, "file or folder exists?"=w317:bool)  [unwired: 8 in, 1 out]
        n143 = case shown="False" w317 {
          tunnel: w316 -> [w324 w325]
          tunnel: [w323 w325] -> w306
          tunnel: w312 -> [w321 _]
          frame False {
            n144 = call-poly <vilib>:"Write To Spreadsheet File.vi"("append to file? (new file:F)"=FALSE, "1D data"=w321, "file path (dialog if empty)"=w324) -> ("new file path (Not A Path if cancelled)"=w323:path)  [unwired: 5 in]
          }
          frame True {
          }
        }
        n145 = in-place {
          in-place-border: w307 -> [w320]
          in-place-border: w306 -> [w319]
          n146 = in-place-cluster #10(w309) -> ()  [unwired: 2 out]
          n147 = in-place-cluster #10("文件保存信息.温度数据保存文件-时间"=w320, "文件保存信息.BasePath"=w319) -> (w308:T8)
        }
      }
      frame "Save: Save" {
        # "#CSM \"Internal State\"\nThis category is used for holding internal states"
        n148 = Unbundle By Name(w326) -> ("State"=w334:T4)
        n149 = Get Date/Time In Seconds() -> (seconds since 1Jan1904=w327:timestamp)
        n150 = call "时间转Excel数字.vi"("温湿度采集时刻"=w327) -> ("数值"=w328:dbl)  [unwired: 10 in]
        n151 = case shown="\"Saving\"" w334 {
          tunnel: [w336 w344 w362] -> w332
          tunnel: w333 -> [w336 w344 w362]
          tunnel: w326 -> [w335 w338 w361]
          tunnel: [w335 w339 w361] -> w329
          tunnel: w328 -> [_ w342 _]
          tunnel: w327 -> [_ w337 _]
          frame "Idle" {
            # "Ignore \"Acquire\" messages when the acquisition is idle."
          }
          frame "Saving" {
            # "Acquire more data while in the \"Acquiring\" state."
            n152 = Unbundle By Name(w338) -> ("数据及Titles.温度相关数据"=w341:T7, "文件保存信息.BasePath"=w340:path)
            n153 = global write "辅助系统全局变量 - T1.vi" "温度相关数据"(w341) -> ()
            n154 = Unbundle By Name(w341) -> ("温度采集"=w345:dbl[], "温度控制"=w346:dbl[], "压力测量"=w347:dbl[], "Zolix"=w348:dbl[], "步进电机"=w343:dbl[], "湿度测量"=w349:dbl[])
            n155 = Build Array (concatenate)(w345, w346, w347, w348, w343, w349) -> (w352:dbl[])
            n156 = Build Array (concatenate)(w342, w352) -> (w353:dbl[])
            n157 = Add Array Elements(numeric array=w352) -> (sum=w350:dbl)
            n158 = Equal To 0?(x=w350) -> (x = 0?=w351:bool)
            n159 = case shown="False" w351 {
              tunnel: w340 -> [w358 w360]
              tunnel: w353 -> [w357 _]
              tunnel: [w355 w360] -> _
              frame False {
                n160 = call-poly <vilib>:"Write To Spreadsheet File.vi"("format (%.3f)"="%.8f", "append to file? (new file:F)"=TRUE, "1D data"=w357, "file path (dialog if empty)"=w358) -> ("new file path (Not A Path if cancelled)"=w355:path)  [unwired: 4 in]
              }
              frame True {
              }
            }
            n161 = in-place {
              in-place-border: w337 -> [w354]
              n162 = in-place-cluster #11(w338) -> ()  [unwired: 1 out]
              n163 = in-place-cluster #11("自停标志.采集时间"=w354) -> (w339:T8)
            }
          }
          frame "Error" {
          }
        }
        n164 = call <vilib>:"Add State(s) to Queue__jki_lib_state_machine.vi"("State(s) in (\"\")"=w330) -> ("States Out"=w331:string)  [unwired: 14 in]
      }
      frame "Save: Stop" {
        # "#CSM \"Internal State\"\nThis category is used for holding internal states"
        n165 = call <vilib>:"Add State(s) to Queue__JKI_lib_State_Machine.vi"("State(s) in (\"\")"=w365) -> ("States Out"=w364:string)  [unwired: 14 in]
      }
      frame "Save: Close" {
        w368 = Saving_States."Idle"  # State
        # "#CSM \"Internal State\"\nThis category is used for holding internal states"
        n166 = in-place {
          in-place-border: w368 -> [w371]
          n167 = in-place-cluster #12(w367) -> ()  [unwired: 1 out]
          n168 = in-place-cluster #12("State"=w371) -> (w366:T8)
        }
        n169 = call <vilib>:"Add State(s) to Queue__JKI_lib_State_Machine.vi"("State(s) in (\"\")"=w370) -> ("States Out"=w369:string)  [unwired: 14 in]
      }
      frame "---------- Loop ----------" {
        # "#CSM \"Internal State\"\nThis category is used for holding internal states"
        n170 = call <vilib>:"Add State(s) to Queue__JKI_lib_State_Machine.vi"("State(s) in (\"\")"=w374) -> ("States Out"=w373:string)  [unwired: 14 in]
      }
      frame "Continuous Check" {
        # "#CSM \"Internal State\"\nThis category is used for holding internal states"
        n171 = Unbundle By Name(w378) -> ("自停标志.接收数"=w395:u32, "自停标志.停止次数"=w392:u32, "自停标志.interval 备份"=w386:dbl, "文件保存信息.Intervals"=w379:dbl, "自停标志.采集时间"=w380:timestamp)
        n172 = Get Date/Time In Seconds() -> (seconds since 1Jan1904=w384:timestamp)
        n173 = feedback-in #13(w395) -> ()
        n174 = feedback #13(u32 0 ("广播数")) -> (w397:u32)
        n175 = Multiply(x=u32 1000 ("y"), y=w379) -> (x*y=w383:dbl)
        n176 = Subtract(x=w384, y=w380) -> (x-y=w382:dbl)
        n177 = Not Equal?(x=w397, y=w395) -> (x != y?=w394:bool)
        n178 = Increment(x=w392) -> (x+1=w391:u32)
        n179 = Divide(x=u32 60, y=w379) -> (x/y=w389:dbl)
        n180 = Subtract(x=w383, y=w382) -> (x-y=w381:dbl)
        n181 = Select(t=u32 0 ("广播数"), s=w394, f=w391) -> (s? t:f=w376:u32)
        n182 = Greater?(x=w391, y=w389) -> (0:w388:bool)
        n183 = Wait (ms)(milliseconds to wait=w381) -> ()  [unwired: 1 out]
        n184 = Select(t=10.0, s=w388, f=w386) -> (s? t:f=w375:dbl)
        n185 = in-place {
          in-place-border: w376 -> [w403]
          in-place-border: w375 -> [w402]
          n186 = in-place-cluster #14(w378) -> ()  [unwired: 2 out]
          n187 = in-place-cluster #14("自停标志.停止次数"=w403, "文件保存信息.Intervals"=w402) -> (w377:T8)
        }
        n188 = call <userlib>:"CSMLS - Append Continuous State.vi"("Loop State(s) And Arguments"=w398, "Continous Arguments (\"\")"=w398, "Continous State"=w400, "States Queue"=w401) -> ("Remaining States"=w399:string)  [unwired: 7 in]
      }
      frame "Break Continuous" {
        n189 = call <userlib>:"CSMLS - Remove Loop Tag to Break.vi"("States Queue"=w406) -> ("Remaining States"=w404:string)  [unwired: 10 in]
      }
    }
  }
  n190 = disable-structure shown="Default" {
    frame condition #0 (active) {
      # "#CSM Check If topmost VI\nSkip the Event Structure if used as subVI"
      # "#CSM Debug User Event\n(No-Event Template Only)\nStop by posting \"Macro: Exit\" Message to lower CSM module. Remove this code after dropping the module to your block diagram. \n\n(delete if after module is tested)"
      n191 = Call Chain() -> (call chain=w409:string[])
      n192 = Array Size(array=w409) -> (size(s)=w408:i32)
      n193 = case shown="1" w408 {
        frame Default {
        }
        frame 1 {
          n194 = event shown="[1] \"Exit\": 值改变" {
            selector: _ -> [_ _]
            dyn-events: _ -> [_ _]
            timeout: _ -> [_ _]
            event Timeout {
              n195 = event-data() -> ()  [unwired: 1 in, 3 out]
            }
            event "Exit": Value Change {
              n196 = event-data() -> ()  [unwired: 1 in, 3 out]
              n197 = local read "CSM Name"() -> (w411:string)
              n198 = call <userlib>:"CSM - Post Message.vi"("Target Module"=w411, "State"="Macro: Exit" ("States")) -> ()  [unwired: 9 in, 1 out]
            }
          }
        }
      }
    }
    frame condition #1 {
    }
  }
